vi "Trade Stock.vi"(7 "sell?":bool, 8 "error in":errorcluster, 9 "quantity":i32=1, 10 "stock name":string, 11 "market":T2) -> (0 "error out":errorcluster, 2 "order":T1, 3 "market out":T2)   [LabVIEW 2020, in "Full Featured MCP Server.lvlib"]
doc: "Buys or sells shares at the current price and returns the new market state and what was traded. An order that cannot be carried out (unknown stock, quantity below 1, not enough money, not enough shares) changes nothing and comes back as error 5100 whose text says what is wrong, so the tool result is marked isError and the assistant can correct itself."
uses:
  Full Featured MCP Server.lvlib
  Market State.ctl
  News Item.ctl
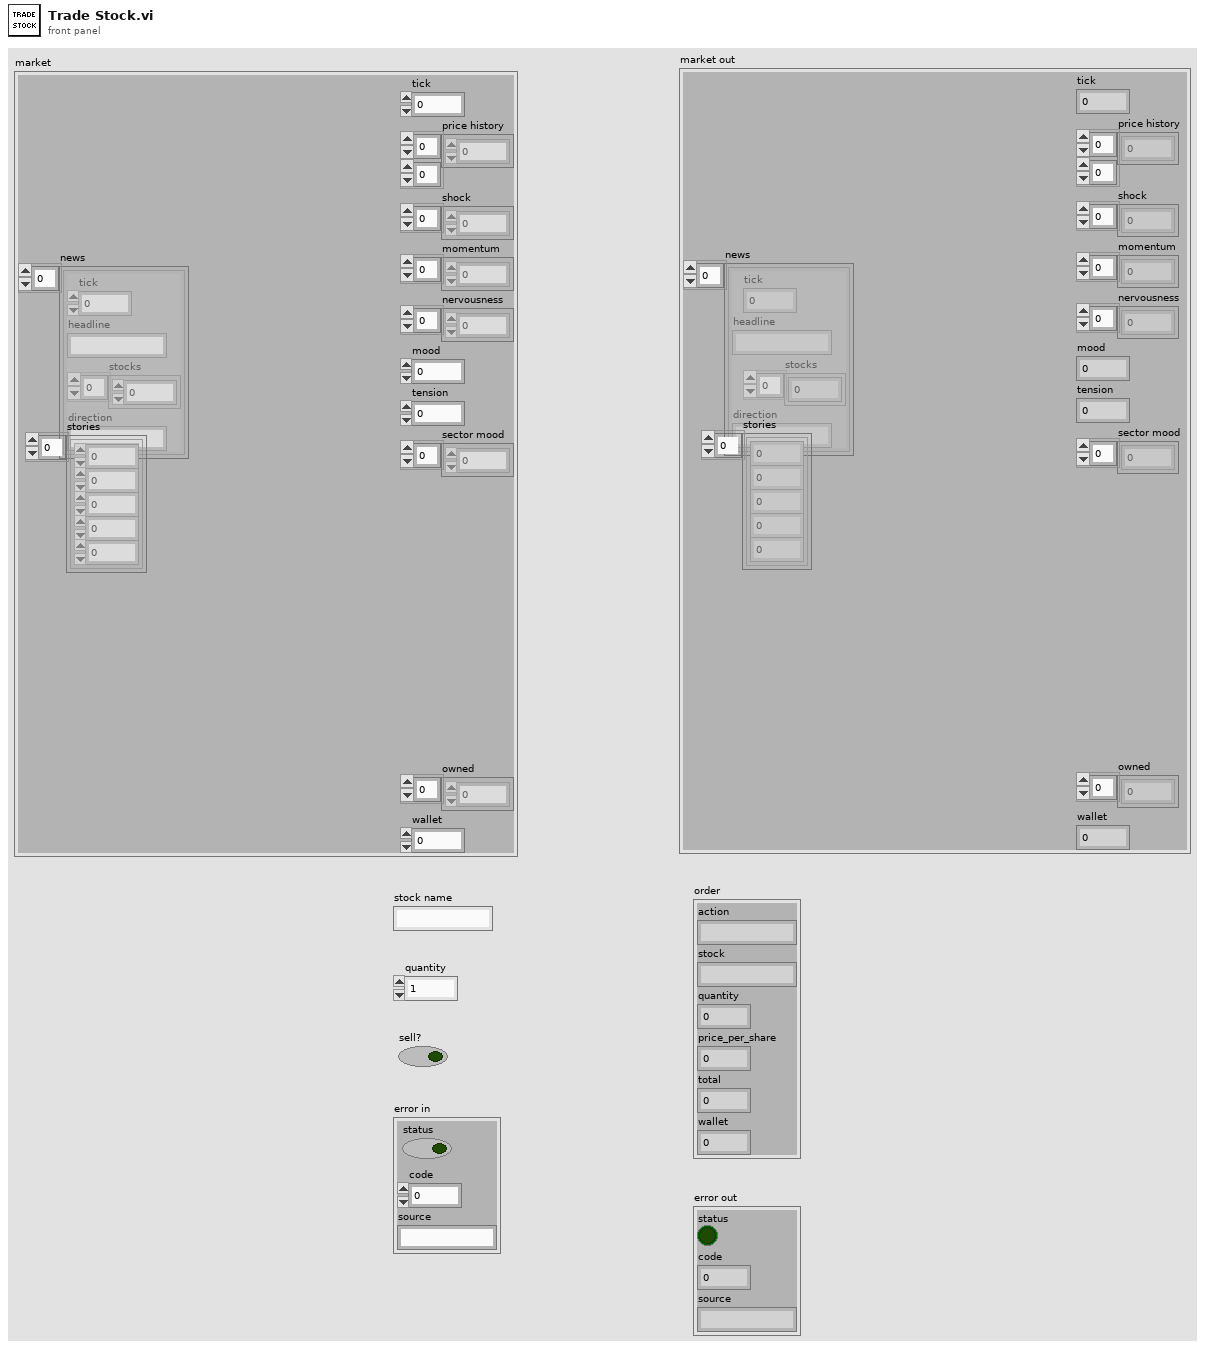
[diagram p1: front panel]
types:
  T1 = cluster{"action":string, "stock":string, "quantity":i32, "price_per_share":dbl, "total":dbl, "wallet":dbl}
  T2 = typedef "Full Featured MCP Server.lvlib/Market State.ctl" = cluster{"tick":i32, "price history":dbl[][], "shock":dbl[], "momentum":dbl[], "nervousness":dbl[], "mood":dbl, "tension":dbl, "sector mood":dbl[], "news":T3[], "stories":cluster{"arc":i32, "step":i32, "due":i32, "stock":i32, "other":i32}[], "owned":i32[], "wallet":dbl}
  T3 = typedef "Full Featured MCP Server.lvlib/News Item.ctl" = cluster{"tick":i32, "headline":string, "stocks":i32[], "direction":string}
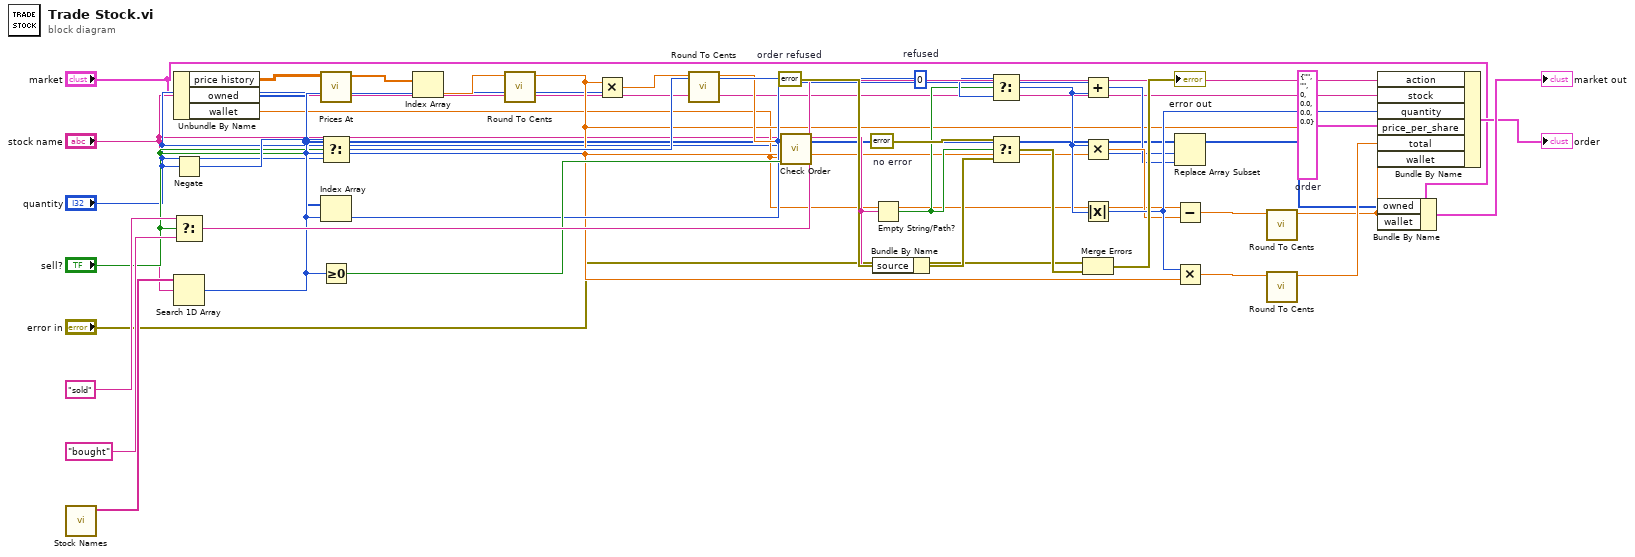
[diagram p0: block diagram]
diagram:
  w39 = errorcluster {"status"=FALSE, "code"=0, "source"=""}  # no error
  w37 = errorcluster {"status"=TRUE, "code"=5100, "source"=""}  # order refused
  w30 = T1 {"action"="", "stock"="", "quantity"=0, "price_per_share"=0.0, "total"=0.0, "wallet"=0.0}  # order
  w22 = 0  # refused
  n1 = call "Stock Names.vi"() -> ("names"=w9:string[])  [unwired: 11 in]
  n2 = Unbundle By Name("market") -> ("price history"=w6:dbl[][], "owned"=w7:i32[], "wallet"=w8:dbl)
  n3 = Negate(x="quantity") -> (-x=w20:i32)
  n4 = Select(t="sold", s="sell?", f="bought") -> (s? t:f=w33:string)
  n5 = Search 1D Array(1D array=w9, element="stock name") -> (index of element=w10:i32)  [unwired: 1 in]
  n6 = call "Prices At.vi"("price history"=w6) -> ("prices"=w11:dbl[])  [unwired: 10 in]
  n7 = Select(t=w20, s="sell?", f="quantity") -> (s? t:f=w21:i32)
  n8 = Index Array(array=w7, index=w10) -> (element=w14:i32)
  n9 = Greater Or Equal To 0?(x=w10) -> (x >= 0?=w17:bool)
  n10 = Index Array(array=w11, index=w10) -> (element=w12:dbl)
  n11 = call "Round To Cents.vi"("amount"=w12) -> ("rounded"=w13:dbl)  [unwired: 10 in]
  n12 = Multiply(x=w13, y="quantity") -> (x*y=w15:dbl)
  n13 = call "Round To Cents.vi"("amount"=w15) -> ("rounded"=w16:dbl)  [unwired: 10 in]
  n14 = call "Check Order.vi"("owned"=w14, "wallet"=w8, "total"=w16, "known?"=w17, "sell?"="sell?", "quantity"="quantity", "stock name"="stock name") -> ("refusal"=w18:string)  [unwired: 4 in]
  n15 = Empty String/Path?(string/path=w18) -> (empty?=w19:bool)
  n16 = Bundle By Name(cluster=w37, "source"=w18) -> (w38:errorcluster)
  n17 = Select(t=w21, s=w19, f=w22) -> (s? t:f=w23:i32)
  n18 = Select(t=w39, s=w19, f=w38) -> (s? t:f=w40:errorcluster)
  n19 = Add(x=w14, y=w23) -> (x+y=w24:i32)
  n20 = Multiply(x=w23, y=w13) -> (x*y=w26:dbl)
  n21 = Absolute Value(x=w23) -> (abs(x)=w29:i32)
  n22 = Merge Errors("error in", w40) -> (→"error out":errorcluster)
  n23 = Replace Array Subset(array=w7, new element=w24, index=w10) -> (w25:i32[])
  n24 = Subtract(x=w8, y=w26) -> (x-y=w27:dbl)
  n25 = Multiply(x=w29, y=w13) -> (x*y=w34:dbl)
  n26 = call "Round To Cents.vi"("amount"=w27) -> ("rounded"=w28:dbl)  [unwired: 10 in]
  n27 = call "Round To Cents.vi"("amount"=w34) -> ("rounded"=w35:dbl)  [unwired: 10 in]
  n28 = Bundle By Name(cluster=w30, "action"=w33, "stock"="stock name", "quantity"=w29, "price_per_share"=w13, "total"=w35, "wallet"=w28) -> (→"order":T1)
  n29 = Bundle By Name(cluster="market", "owned"=w25, "wallet"=w28) -> (→"market out":T2)
